vi "Test Popup API.vi"() -> ()   [LabVIEW 2018]
doc: "Popup API Tester."
uses:
  <vilib>/MGI/Panel Manager/Panel/Panel/Window/Window.lvclass
  C:/Program Files (x86)/National Instruments/LabVIEW 2018/vi.lib/MGI/Panel Manager/Panel/Panel/Panel.lvclass
  <vilib>/MGI/Panel Manager/Panel/Panel/Window/Dialog/Dialog.lvclass
  <vilib>/MGI/Panel Manager/Panel/Panel/Subpanel/Subpanel.lvclass
  <vilib>/MGI/Panel Manager/Panel/Panel/Window/Window.vi
  <vilib>/MGI/Panel Manager/Panel/Panel/Window/Dialog/Dialog.vi
  <vilib>/MGI/Panel Manager/Panel/Panel/Subpanel/Subpanel.vi
  Popup.lvlib
  <vilib>/MGI/Panel Manager/Panel/Panel.lvlib
panel:
  in  "标题":string
  in  "Modify Title name":bool
  in  "Right":i16
  in  "Bottom":i16
  in  "Left":i16
  in  "Top":i16
  in  "Modify window front":bool
  in  "Origin":cluster{"Horizontal":i16, "Vertical":i16}
  in  "modify panl  origin position":bool
  in  "Autoshow?":bool
  in  "Panel Type":enum16{"Window", "Dialog", "Subpanel"}(ring)
  in  "Change Panel":bool
  in  "Tab Control":enum32{"Status", "Subpanel"}(tab)
  out "Status":string
  in  "Run as Singleton?":bool
  in  "Show Block Diagram":bool
  in  "Refresh Modules":bool
  out "Active Modules":string[](array[string])
  in  "Stop Module":bool
  in  "Select Module":i32(ring)=-1 caption="Select Module\nTo send Request to" items=["All"=-1]
  in  "Run New Module":bool
  in  "Hide Module Panel":bool
  in  "Show Module Panel":bool
  # "This VI tests the API for the Module."
  # "Change Panel"
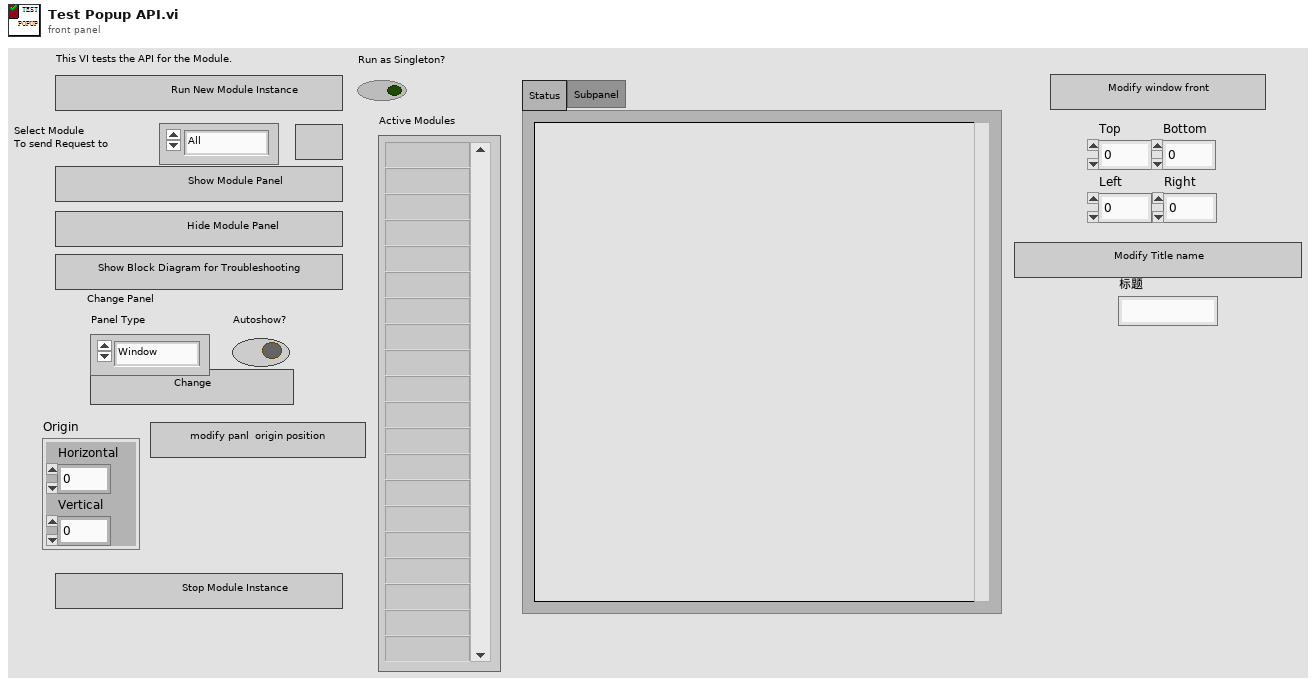
[diagram p1: front panel]
types:
  T1 = typedef "Popup.lvlib/Broadcast Events--cluster.ctl" = cluster{"Module Did Init":refnum<user-event>, "Status Updated":refnum<user-event>, "Error Reported":refnum<user-event>, "Module Did Stop":refnum<user-event>, "Update Module Execution Status":refnum<user-event>}
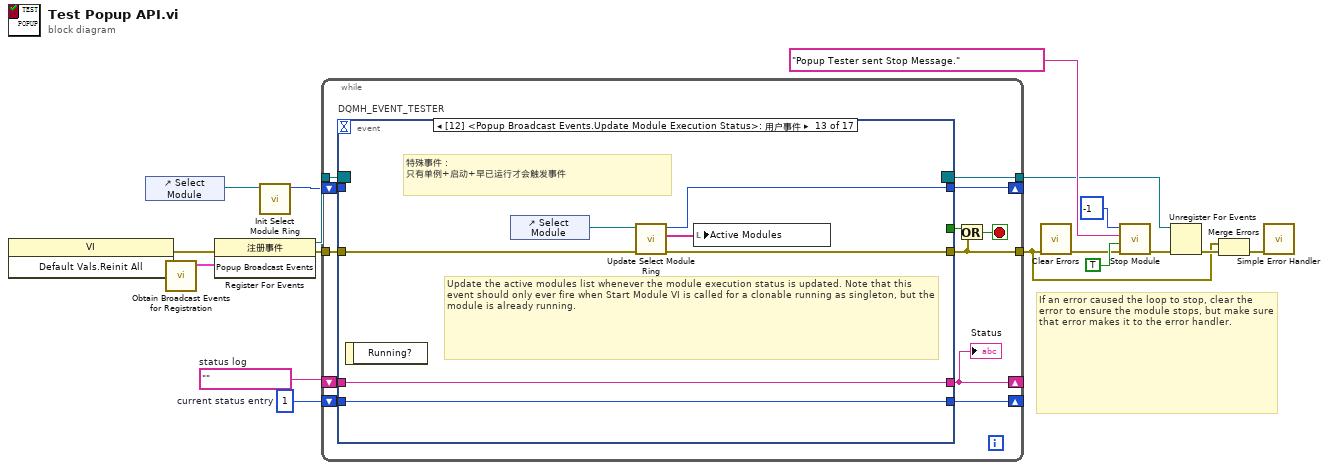
[diagram p0: block diagram]
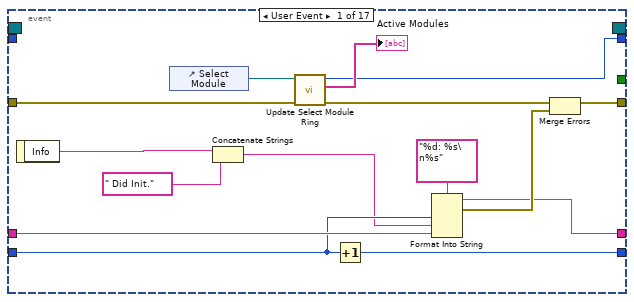
[diagram p2: hidden frame]
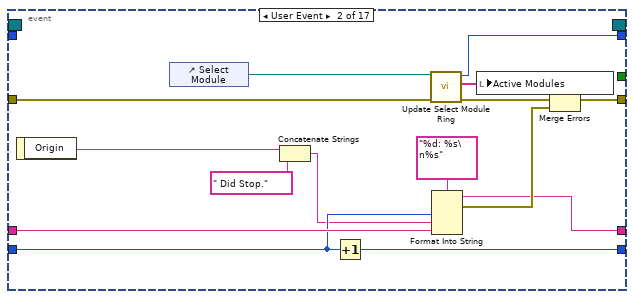
[diagram p3: hidden frame]
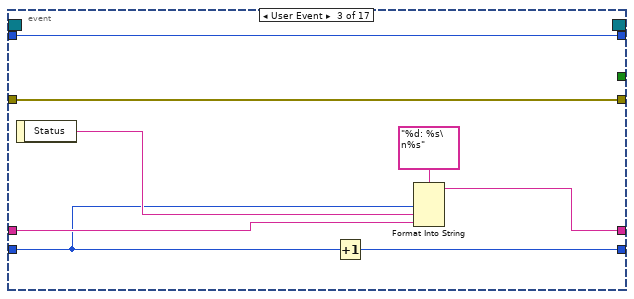
[diagram p4: hidden frame]
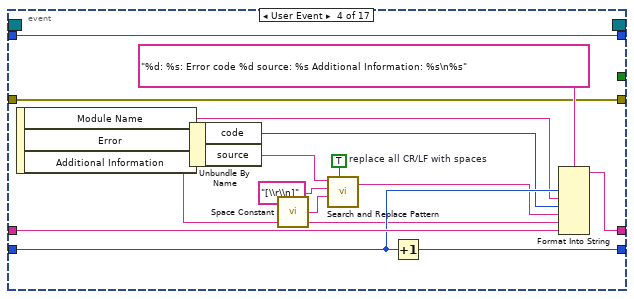
[diagram p5: hidden frame]
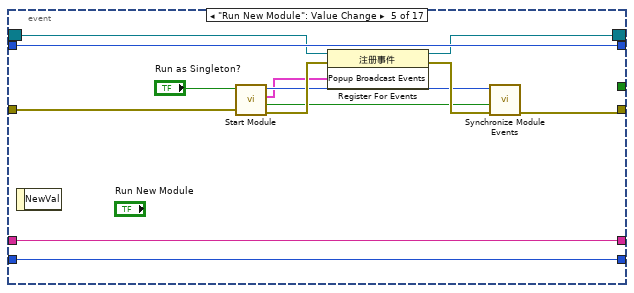
[diagram p6: hidden frame]
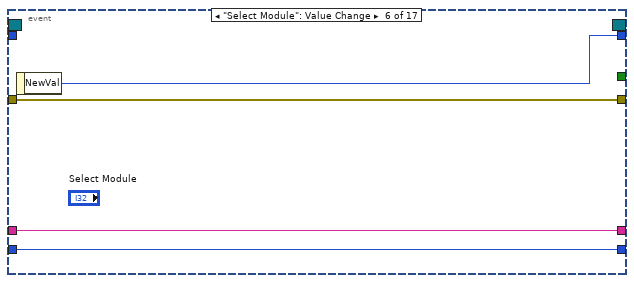
[diagram p7: hidden frame]
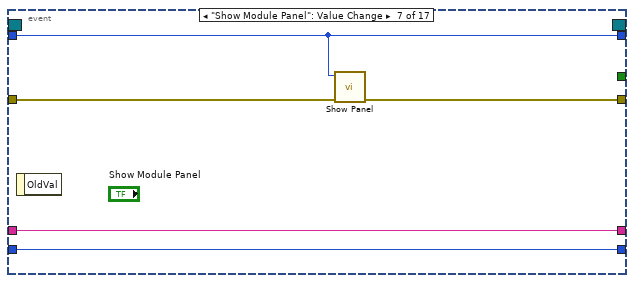
[diagram p8: hidden frame]
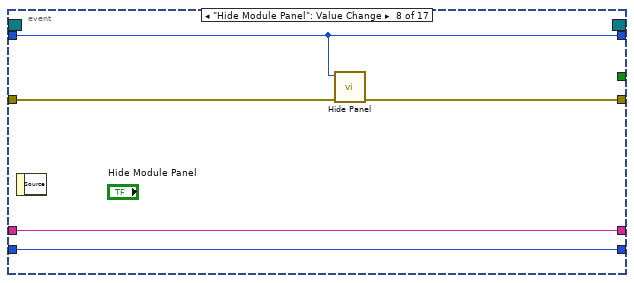
[diagram p9: hidden frame]
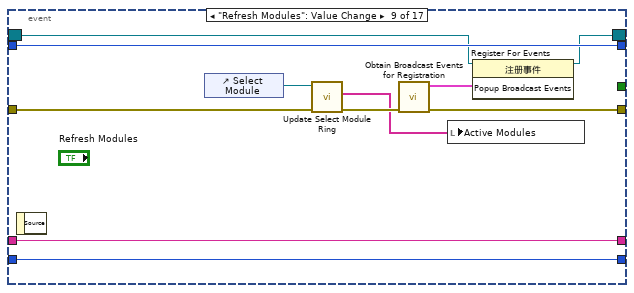
[diagram p10: hidden frame]
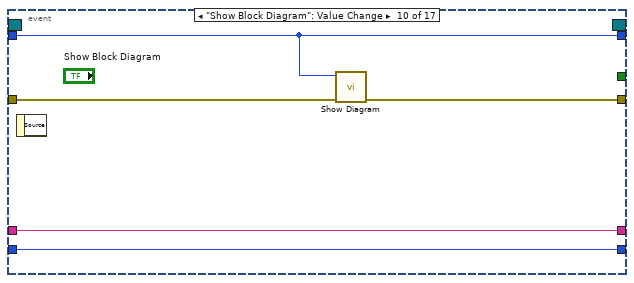
[diagram p11: hidden frame]
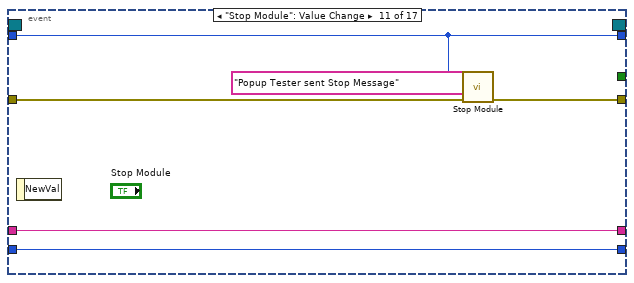
[diagram p12: hidden frame]
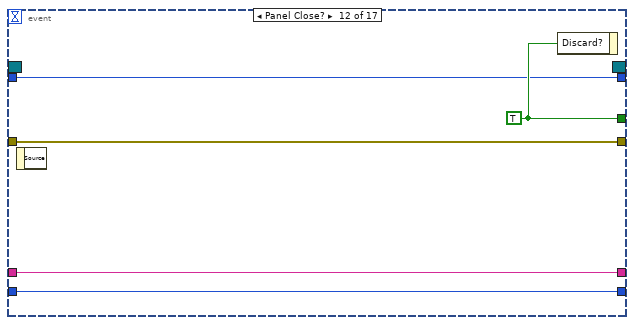
[diagram p13: hidden frame]
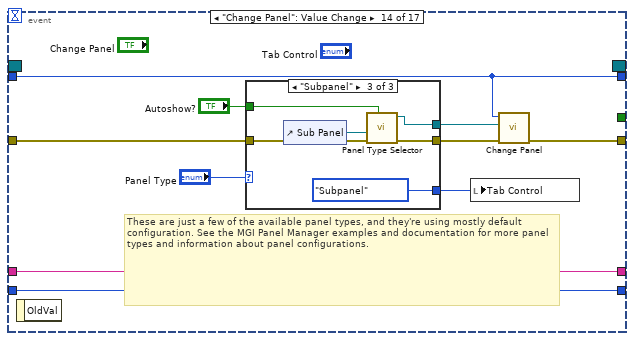
[diagram p14: hidden frame]
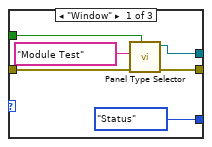
[diagram p15: hidden frame]
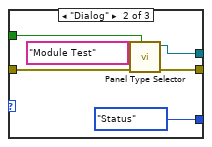
[diagram p16: hidden frame]
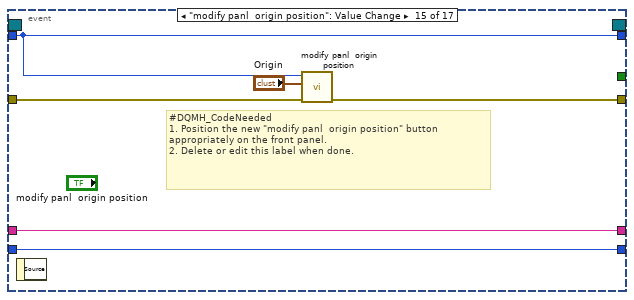
[diagram p17: hidden frame]
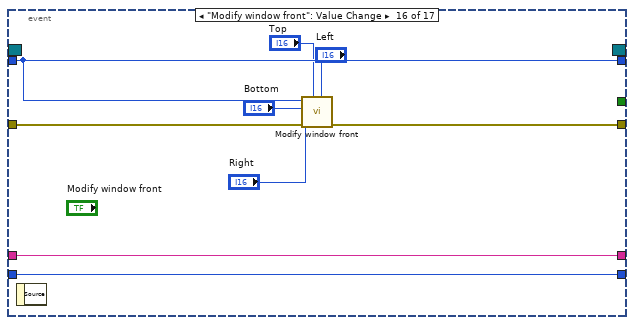
[diagram p18: hidden frame]
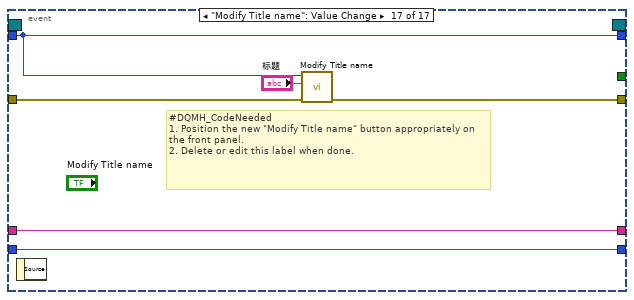
[diagram p19: hidden frame]
diagram:
  w13 = 1  # current status entry
  w14 = ""  # status log
  # "If an error caused the loop to stop, clear the error to ensure the module stops, but make sure that error makes it to the error handler."
  n1 = invoke class="VI" method="Default Vals.Reinit All"() -> (error out=w6:errorcluster)  [unwired: 3 in, 2 out]
  n2 = control-ref of="Select Module"() -> (w11:refnum<vi>)
  n3 = call "Obtain Broadcast Events for Registration.vi"() -> ("Popup Broadcast Events"=w10:T1)  [unwired: 10 in, 1 out]
  n4 = register-events(error in=w6, w10) -> (reference out=w17:refnum<event-registration>, error out=w9:errorcluster)  [unwired: 1 in]
  n5 = call "Init Select Module Ring.vi"("Select Module Ring Ref"=w11) -> ("Value for All Modules"=w12:i32)  [unwired: 8 in, 2 out]
  n6 = while {
    tunnel: w17 -> [w29]
    tunnel: [w18] -> w1
    tunnel: w9 -> [w27]
    shift-right: [w23] -> _
    shift-left: w14 -> [w25]
    shift-right: [w24] -> _
    shift-left: w13 -> [w26]
    shift-right: [w20] -> _
    shift-left: w12 -> [w21]
    tunnel: [w19] -> w5
    stop <- w22 stop-if-true
    n7 = event "DQMH_EVENT_TESTER" shown="[12] <Popup Broadcast Events.Update Module Execution Status>: 用户事件" {
      selector: w29 -> [_ _ _ _ w91 _ _ _ w116 _ _ _ _ _ _ _ _]
      dyn-events: [_ _ _ _ w90 _ _ _ w115 _ _ _ _ _ _ _ _] -> w19
      timeout: _ -> [_ _ _ _ _ _ _ _ _ _ _ _ _ _ _ _ _]
      tunnel: [_ _ _ _ _ _ _ _ _ _ _ w137 _ _ _ _ _] -> w28
      tunnel: [w33 w51 w67 w73 w89 w100 w104 w109 w112 w123 w128 w136 w140 w152 w174 w183 w189] -> w18
      tunnel: w27 -> [w35 w53 w67 w73 w84 w100 w105 w110 w117 w126 w129 w136 w141 w148 w178 w187 w193]
      tunnel: w26 -> [w41 w56 w60 w79 w93 w98 w102 w107 w120 w124 w131 w134 w143 w153 w176 w185 w191]
      tunnel: w25 -> [w42 w57 w63 w81 w94 w99 w103 w108 w121 w125 w132 w135 w144 w154 w177 w186 w192]
      tunnel: [w39 w54 w64 w76 w94 w99 w103 w108 w121 w125 w132 w135 w144 w154 w177 w186 w192] -> w23
      tunnel: [w40 w55 w66 w82 w93 w98 w102 w107 w120 w124 w131 w134 w143 w153 w176 w185 w191] -> w24
      tunnel: w21 -> [_ _ w61 w83 w92 _ w101 w106 w119 w122 w130 w133 _ w151 w175 w184 w190]
      tunnel: [w30 w48 w61 w83 w92 w97 w101 w106 w119 w122 w130 w133 w139 w151 w175 w184 w190] -> w20
      event User Event {
        n8 = event-data() -> ("Info"=w38:string)  [unwired: 1 in]
        n9 = control-ref of="Select Module"() -> (w32:refnum<vi>)
        n10 = Concatenate Strings(w38, " Did Init.") -> (w37:string)
        n11 = call "Update Select Module Ring.vi"("error in (no error)"=w35, "Select Module Ring Ref"=w32) -> ("error out"=w34:errorcluster, "Active Modules (Array)"=→"Active Modules":string[], "New Module Ring Value"=w30:i32)  [unwired: 7 in]
        n12 = Increment(x=w41) -> (x+1=w40:i32)
        n13 = Format Into String(format string="%d: %s\n%s", w41, w37, w42) -> (resulting string=w39:string, error out=w44:errorcluster)  [unwired: 2 in]
        n14 = Merge Errors(w34, w44) -> (w33:errorcluster)
      }
      event User Event {
        n15 = event-data() -> ("Origin"=w46:string)  [unwired: 1 in]
        n16 = control-ref of="Select Module"() -> (w50:refnum<vi>)
        n17 = Concatenate Strings(w46, " Did Stop.") -> (w45:string)
        n18 = Increment(x=w56) -> (x+1=w55:i32)
        n19 = call "Update Select Module Ring.vi"("error in (no error)"=w53, "Select Module Ring Ref"=w50) -> ("error out"=w52:errorcluster, "Active Modules (Array)"=w49:string[], "New Module Ring Value"=w48:i32)  [unwired: 7 in]
        n20 = Format Into String(format string="%d: %s\n%s", w56, w45, w57) -> (resulting string=w54:string, error out=w59:errorcluster)  [unwired: 2 in]
        n21 = local write "Active Modules"(w49) -> ()
        n22 = Merge Errors(w52, w59) -> (w51:errorcluster)
      }
      event User Event {
        n23 = event-data() -> ("Status"=w62:string)  [unwired: 1 in]
        n24 = Increment(x=w60) -> (x+1=w66:i32)
        n25 = Format Into String(format string="%d: %s\n%s", w60, w62, w63) -> (resulting string=w64:string)  [unwired: 2 in, 1 out]
      }
      event User Event {
        w77 = TRUE  # replace all CR/LF with spaces
        n26 = event-data() -> ("Module Name"=w71:string, "Error"=w70:errorcluster, "Additional Information"=w68:string)  [unwired: 1 in]
        n27 = Unbundle By Name(w70) -> ("code"=w72:i32, "source"=w74:string)
        n28 = call <vilib>:"Space Constant.vi"() -> ("String"=w78:string)
        n29 = call <vilib>:"Search and Replace Pattern.vi"("string"=w74, "regular expression (\"\")"="[\\r\\n]" ("regular expression (\"\")"), "replace string (\"\")"=w78, "replace all? (F)"=w77) -> ("result string"=w75:string)  [unwired: 1 in, 1 out]
        n30 = Increment(x=w79) -> (x+1=w82:i32)
        n31 = Format Into String(format string="%d: %s: Error code %d source: %s Additional Information: %s\n%s", w79, w71, w72, w75, w68, w81) -> (resulting string=w76:string)  [unwired: 2 in, 1 out]
      }
      event "Run New Module": Value Change {
        n32 = event-data() -> ()  [unwired: 1 in, 1 out]
        n33 = call "Start Module.vi"("error in (no error)"=w84, "Run as Singleton? (F)"="Run as Singleton?") -> ("error out"=w95:errorcluster, "Wait for Event Sync?"=w87:bool, "Popup Broadcast Events"=w86:T1, "Module ID"=w88:i32)  [unwired: 6 in]
        n34 = register-events(reference=w91, error in=w95, w86) -> (reference out=w90:refnum<event-registration>, error out=w96:errorcluster)
        n35 = call "Synchronize Module Events.vi"("error in (no error)"=w96, "Wait for Event Sync?"=w87, "Module ID"=w88) -> ("error out"=w89:errorcluster)  [unwired: 7 in, 1 out]
      }
      event "Select Module": Value Change {
        n36 = event-data() -> ("NewVal"=w97:i32)  [unwired: 1 in]
      }
      event "Show Module Panel": Value Change {
        n37 = event-data() -> ()  [unwired: 1 in, 1 out]
        n38 = call "Show Panel.vi"("error in (no error)"=w105, "Module ID"=w101) -> ("error out"=w104:errorcluster)  [unwired: 9 in]
      }
      event "Hide Module Panel": Value Change {
        n39 = event-data() -> ()  [unwired: 1 in, 1 out]
        n40 = call "Hide Panel.vi"("error in (no error)"=w110, "Module ID"=w106) -> ("error out"=w109:errorcluster)  [unwired: 9 in]
      }
      event "Refresh Modules": Value Change {
        n41 = event-data() -> ()  [unwired: 1 in, 1 out]
        n42 = control-ref of="Select Module"() -> (w118:refnum<vi>)
        n43 = call "Update Select Module Ring.vi"("error in (no error)"=w117, "Select Module Ring Ref"=w118) -> ("error out"=w113:errorcluster, "Active Modules (Array)"=w111:string[])  [unwired: 7 in, 1 out]
        n44 = call "Obtain Broadcast Events for Registration.vi"("error in (no error)"=w113) -> ("error out"=w112:errorcluster, "Popup Broadcast Events"=w114:T1)  [unwired: 9 in]
        n45 = local write "Active Modules"(w111) -> ()
        n46 = register-events(reference=w116, w114) -> (reference out=w115:refnum<event-registration>)  [unwired: 1 in, 1 out]
      }
      event "Show Block Diagram": Value Change {
        n47 = event-data() -> ()  [unwired: 1 in, 1 out]
        n48 = call "Show Diagram.vi"("error in (no error)"=w126, "Module ID"=w122) -> ("error out"=w123:errorcluster)  [unwired: 9 in]
      }
      event "Stop Module": Value Change {
        n49 = event-data() -> ()  [unwired: 1 in, 1 out]
        n50 = call "Stop Module.vi"("error in (no error)"=w129, "Origin"="Popup Tester sent Stop Message", "Module ID"=w130) -> ("error out"=w128:errorcluster)  [unwired: 8 in]
      }
      event Panel Close? {
        w137 = TRUE ("Discard?")
        n51 = event-data() -> ()  [unwired: 1 in, 1 out]
        n52 = event-data("Discard?"=w137) -> ()  [unwired: 1 in, 1 out]
      }
      event User Event {
        # "特殊事件：\n只有单例+启动+早已运行才会触发事件"
        # "Update the active modules list whenever the module execution status is updated. Note that this event should only ever fire when Start Module VI is called for a clonable running as singleton, but the module is already running."
        n53 = event-data() -> ()  [unwired: 1 in, 1 out]
        n54 = control-ref of="Select Module"() -> (w142:refnum<vi>)
        n55 = call "Update Select Module Ring.vi"("error in (no error)"=w141, "Select Module Ring Ref"=w142) -> ("error out"=w140:errorcluster, "Active Modules (Array)"=w138:string[], "New Module Ring Value"=w139:i32)  [unwired: 7 in]
        n56 = local write "Active Modules"(w138) -> ()
      }
      event "Change Panel": Value Change {
        # "These are just a few of the available panel types, and they're using mostly default configuration. See the MGI Panel Manager examples and documentation for more panel types and information about panel configurations."
        n57 = event-data() -> ()  [unwired: 1 in, 1 out]
        n58 = case shown="\"Subpanel\"" "Panel Type" {
          tunnel: [w160 w166 w172] -> w150
          tunnel: [w159 w165 w171] -> w149
          tunnel: w148 -> [w157 w163 w170]
          tunnel: [enum32{"Status", "Subpanel"}."Status" ("Tab Control") enum32{"Status", "Subpanel"}."Status" ("Tab Control") enum32{"Status", "Subpanel"}."Subpanel" ("Tab Control")] -> w147
          tunnel: "Autoshow?" -> [w155 w161 w168]
          frame "Window" {
            n59 = call-poly <vilib>:"Panel Type Selector.vi"("Autoshow? (T)"=w155, "error in (no error)"=w157, "Default Title"="Module Test") -> ("error out"=w159:errorcluster, "Window out"=w160:refnum<class "Window.lvclass">)  [unwired: 7 in]
          }
          frame "Dialog" {
            n60 = call-poly <vilib>:"Panel Type Selector.vi"("Autoshow? (T)"=w161, "Error In"=w163, "Default Title"="Module Test") -> ("Error Out"=w165:errorcluster, "Dialog out"=w166:refnum<class "Dialog.lvclass">)  [unwired: 7 in]
          }
          frame "Subpanel" {
            n61 = control-ref of="Sub Panel"() -> (w167:refnum<vi>)
            n62 = call-poly <vilib>:"Panel Type Selector.vi"("Autoshow? (T)"=w168, "Error In"=w170, "Sub Panel"=w167) -> ("Error Out"=w171:errorcluster, "Subpanel Out"=w172:refnum<class "Subpanel.lvclass">)  [unwired: 7 in]
          }
        }
        n63 = local write "Tab Control"(w147) -> ()
        n64 = call "Change Panel.vi"("error in (no error)"=w149, "New Panel"=w150, "Module ID"=w151) -> ("error out"=w152:errorcluster)  [unwired: 8 in]
      }
      event "modify panl  origin position": Value Change {
        # "#DQMH_CodeNeeded\n1. Position the new \"modify panl  origin position\" button appropriately on the front panel.\n2. Delete or edit this label when done."
        n65 = event-data() -> ()  [unwired: 1 in, 1 out]
        n66 = call "modify panl  origin position.vi"("error in"=w178, "Origin"="Origin", "Module ID"=w175) -> ("error out"=w174:errorcluster)  [unwired: 8 in]
      }
      event "Modify window front": Value Change {
        n67 = event-data() -> ()  [unwired: 1 in, 1 out]
        n68 = call "Modify window front.vi"("Left"="Left", "Top"="Top", "error in"=w187, "Right"="Right", "Bottom"="Bottom", "Module ID"=w184) -> ("error out"=w183:errorcluster)  [unwired: 5 in]
      }
      event "Modify Title name": Value Change {
        # "#DQMH_CodeNeeded\n1. Position the new \"Modify Title name\" button appropriately on the front panel.\n2. Delete or edit this label when done."
        n69 = event-data() -> ()  [unwired: 1 in, 1 out]
        n70 = call "Modify Title name.vi"("error in"=w193, "标题"="标题", "Module ID"=w190) -> ("error out"=w189:errorcluster)  [unwired: 8 in]
      }
    }
    "Status" <- w23
    n71 = Or(x=w28, y=w18) -> (x .or. y?=w22:bool)
  }
  n72 = call <vilib>:"Clear Errors.vi"("error in (no error)"=w1) -> ("error out"=w3:errorcluster)  [unwired: 5 in, 1 out]
  n73 = call "Stop Module.vi"("error in (no error)"=w3, "Wait for Module to stop? (F)"=TRUE ("Wait for Module to stop?"), "Origin"="Popup Tester sent Stop Message.", "Module ID"=-1 ("Stop all")) -> ("error out"=w15:errorcluster)  [unwired: 7 in]
  n74 = Unregister For Events(event registration refnum=w5, error in=w15) -> (error out=w16:errorcluster)
  n75 = Merge Errors(w1, w16) -> (w2:errorcluster)
  n76 = call <vilib>:"Simple Error Handler.vi"("error in (no error)"=w2) -> ()  [unwired: 4 in, 5 out]
